vi "Host_Actor_Launcher.vi"(8 "error in (no error)":errorcluster={"status"=FALSE, "code"=0, "source"="\"\""}, 9 "Config Path":string="configs/test_profile_sim.json", 10 "Recipe ID":string="RECIPE_SIM_001") -> (0 "error out":errorcluster, 1 "Active Recipe":string, 2 "Actor Launcher Status":string)   [LabVIEW 2026]
doc: "INTENT: Top-level Launcher for Host Actor in Actor Framework architecture."
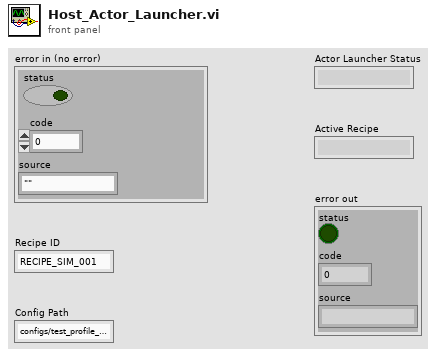
[diagram p1: front panel]
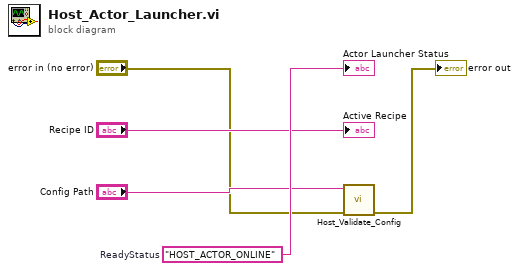
[diagram p0: block diagram]
diagram:
  w5 = "HOST_ACTOR_ONLINE"  # ReadyStatus
  n1 = call "Host_Validate_Config.vi"("error in (no error)"="error in (no error)", "Editable config package"="Config Path") -> ("error out"=→"error out":errorcluster)  [unwired: 7 in, 2 out]
  "Actor Launcher Status" <- w5
  "Active Recipe" <- "Recipe ID"
